vi "Measure the Function on 1st Display.vi"(5 "Type for Temperature":u8(ring) items=["J Type", "K Type", "T Type"], 7 "Manual Range":dbl format="%#.9e", 8 "error in":errorcluster, 9 "Enable Auto Range":bool=TRUE, 10 "Function":u8(ring) items=["DC Voltage", "AC Voltage", "DC Current", "AC Current", "2-Wire Resistance", "4-Wire Resistance", "Frequency", "Period", "Continuity", "Diode", "Temperature", "Capacitance"], 11 "VISA resource name":refnum<visa-resource-name>) -> (0 "error out":errorcluster, 2 "Return the Value":string, 3 "VISA resource name out":refnum<visa-resource-name>)   [LabVIEW 2012, in "GDM-9052.lvlib"]
uses:
  GDM-9052.lvlib
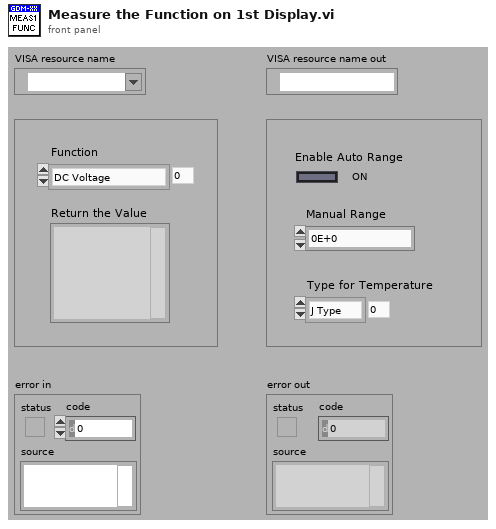
[diagram p1: front panel]
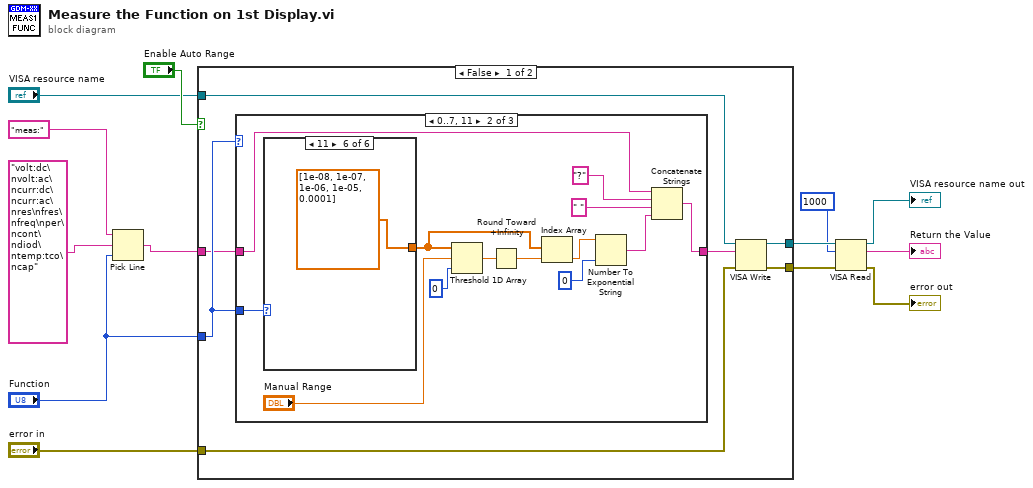
[diagram p0: block diagram]
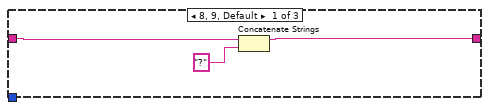
[diagram p2: hidden frame]
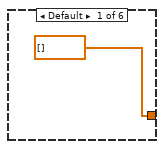
[diagram p3: hidden frame]
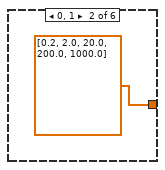
[diagram p4: hidden frame]
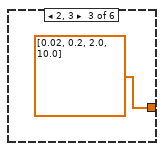
[diagram p5: hidden frame]
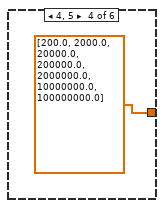
[diagram p6: hidden frame]
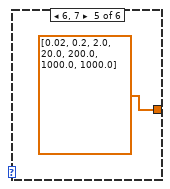
[diagram p7: hidden frame]
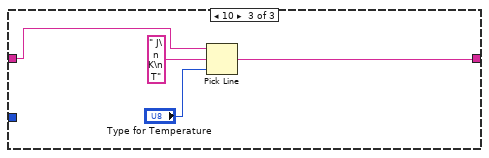
[diagram p8: hidden frame]
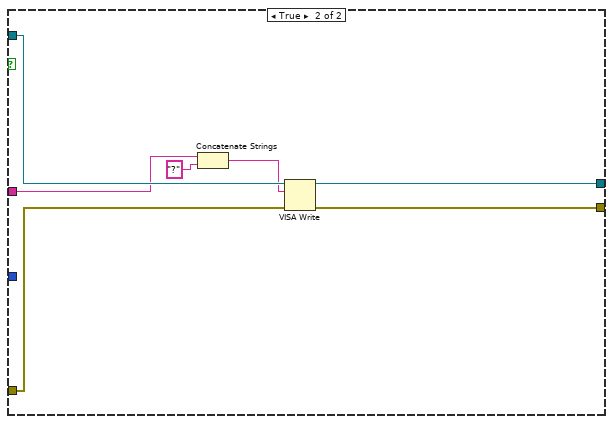
[diagram p9: hidden frame]
diagram:
  n1 = Pick Line(string ("")="meas:", multi-line string="volt:dc\nvolt:ac\ncurr:dc\ncurr:ac\nres\nfres\nfreq\nper\ncont\ndiod\ntemp:tco\ncap", line index="Function") -> (output string=w9:string)
  n2 = case shown="False" "Enable Auto Range" {
    tunnel: "Function" -> [w20 _]
    tunnel: w9 -> [w19 w49]
    tunnel: "VISA resource name" -> [w17 w53]
    tunnel: "error in" -> [w16 w52]
    tunnel: [w15 w51] -> w6
    tunnel: [w14 w50] -> w5
    frame False {
      n3 = case shown="0..7, 11" w20 {
        tunnel: w20 -> [_ w26 _]
        tunnel: w19 -> [w22 w25 w43]
        tunnel: [w21 w27 w44] -> w18
        frame 8, 9, Default {
          n4 = Concatenate Strings(w22, "?" ("string")) -> (w21:string)
        }
        frame 0..7, 11 {
          n5 = case shown="11" w26 {
            tunnel: [dbl[] [] dbl[] [0.2, 2.0, 20.0, 200.0, 1000.0] dbl[] [0.02, 0.2, 2.0, 10.0] dbl[] [200.0, 2000.0, 20000.0, 200000.0, 2000000.0, 10000000.0, 100000000.0] dbl[] [0.02, 0.2, 2.0, 20.0, 200.0, 1000.0, 1000.0] dbl[] [1e-08, 1e-07, 1e-06, 1e-05, 0.0001]] -> w32
            frame Default {
            }
            frame 0, 1 {
            }
            frame 2, 3 {
            }
            frame 4, 5 {
            }
            frame 6, 7 {
            }
            frame 11 {
            }
          }
          n6 = Threshold 1D Array(1:0 ("start index (0)"), 2:"Manual Range", 3:w32) -> (0:w34:dbl)
          n7 = Round Toward +Infinity(x=w34) -> (ceil(x): smallest int >= x=w33:dbl)
          n8 = Index Array(array=w32, index=w33) -> (element=w31:dbl)
          n9 = Number To Exponential String(number=w31, precision (6)=i16 0) -> (E-format string=w28:string)  [unwired: 2 in]
          n10 = Concatenate Strings(w25, "?" ("string"), " " ("string"), w28) -> (w27:string)
        }
        frame 10 {
          n11 = Pick Line(string ("")=w43, multi-line string=" J\n K\n T", line index="Type for Temperature") -> (output string=w44:string)
        }
      }
      n12 = VISA Write(VISA resource name=w17, write buffer=w18, error in (no error)=w16) -> (VISA resource name out=w15:refnum<visa-resource-name>, error out=w14:errorcluster)  [unwired: 1 out]
    }
    frame True {
      n13 = Concatenate Strings(w49, "?" ("string")) -> (w47:string)
      n14 = VISA Write(VISA resource name=w53, write buffer=w47, error in (no error)=w52) -> (VISA resource name out=w51:refnum<visa-resource-name>, error out=w50:errorcluster)  [unwired: 1 out]
    }
  }
  n15 = VISA Read(VISA resource name=w6, byte count=u32 1000, error in (no error)=w5) -> (VISA resource name out=→"VISA resource name out":refnum<visa-resource-name>, read buffer=→"Return the Value":string, error out=→"error out":errorcluster)  [unwired: 1 out]
